vi "Get XNET Signal Names.vi"(6 "Add Info?":bool, 7 "Parent Ref in":T1 format="%.0x", 8 "error in":errorcluster, 9 "Tree In":refnum<vi>, 10 "XNET Cluster":refnum<k21>) -> (0 "error out":errorcluster, 1 "Tree Out":refnum<vi>, 3 "XNET Signal Names":refnum<k21>[](array[refnum]))   [LabVIEW 2025, in "Protection and Counter Addon System Explorer.lvlib"]
uses:
  Protection and Counter Addon System Explorer.lvlib
  <vilib>/NI VeriStand/Custom Device API/Custom Device Item Ref.ctl
  Types/Frame Tree and Database Pairing.ctl
  <vilib>/NI VeriStand/Custom Device API/Custom Device Channel.ctl
  <vilib>/NI VeriStand/Custom Device API/Custom Device Channel Type.ctl
  <vilib>/xnet/xnet.llb/XNET Get DBC Mode.ctl
  Addon Shared/SubVIs/GUID Lookup.vi
  <vilib>/NI VeriStand/Custom Device Tools/Custom Device Utility Library/NI VeriStand - Search for Item by Name.vi
  <vilib>/NI VeriStand/Custom Device API/Set Item Property (U32).vi
  <vilib>/xnet/xnet.llb/XNET Database Get DBC Attribute (Signal).vi
  <resource>/objmgr/xnet.rc
  <vilib>/NI VeriStand/Custom Device API/Custom Device API.lvlib
  Addon Shared/Protection and Counter Addon Shared.lvlib
  <vilib>/NI VeriStand/Custom Device Tools/Custom Device Utility Library/Custom Device Utility Library.lvlib
  <vilib>/NI/NI VeriStand Advanced SysDef API/SysDef API/Advanced System Definition.lvlib
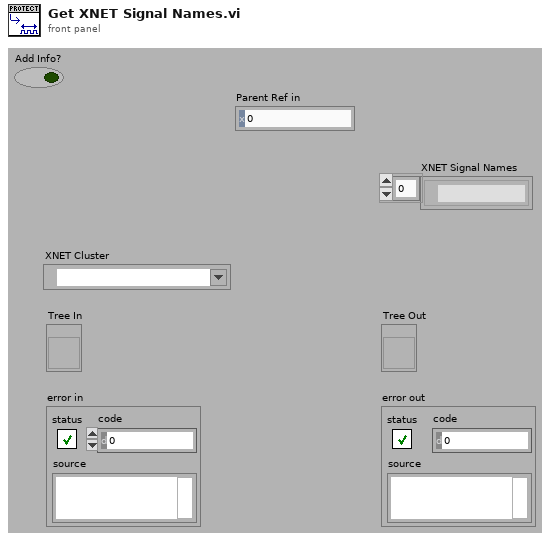
[diagram p1: front panel]
types:
  T1 = typedef "Custom Device API.lvlib/Custom Device Item Ref.ctl" = u64
  T2 = typedef "Protection and Counter Addon System Explorer.lvlib/Frame Tree and Database Pairing.ctl" = cluster{"Tree Tag":string, "Database Tag":string}
  T3 = typedef "Custom Device API.lvlib/Custom Device Channel.ctl" = cluster{"Type":T4, "Units":string, "Default Value":dbl, "Faultable":bool, "Scalable":bool}
  T4 = typedef "Custom Device API.lvlib/Custom Device Channel Type.ctl" = enum16{"Input", "Output"}
  T5 = typedef "Custom Device API.lvlib/Custom Device Item Info.ctl" = cluster{"Name":string, "Is Channel":bool, "GUID":string, "Is Waveform":bool}
  T6 = typedef "XNET Get DBC Mode.ctl" = u32
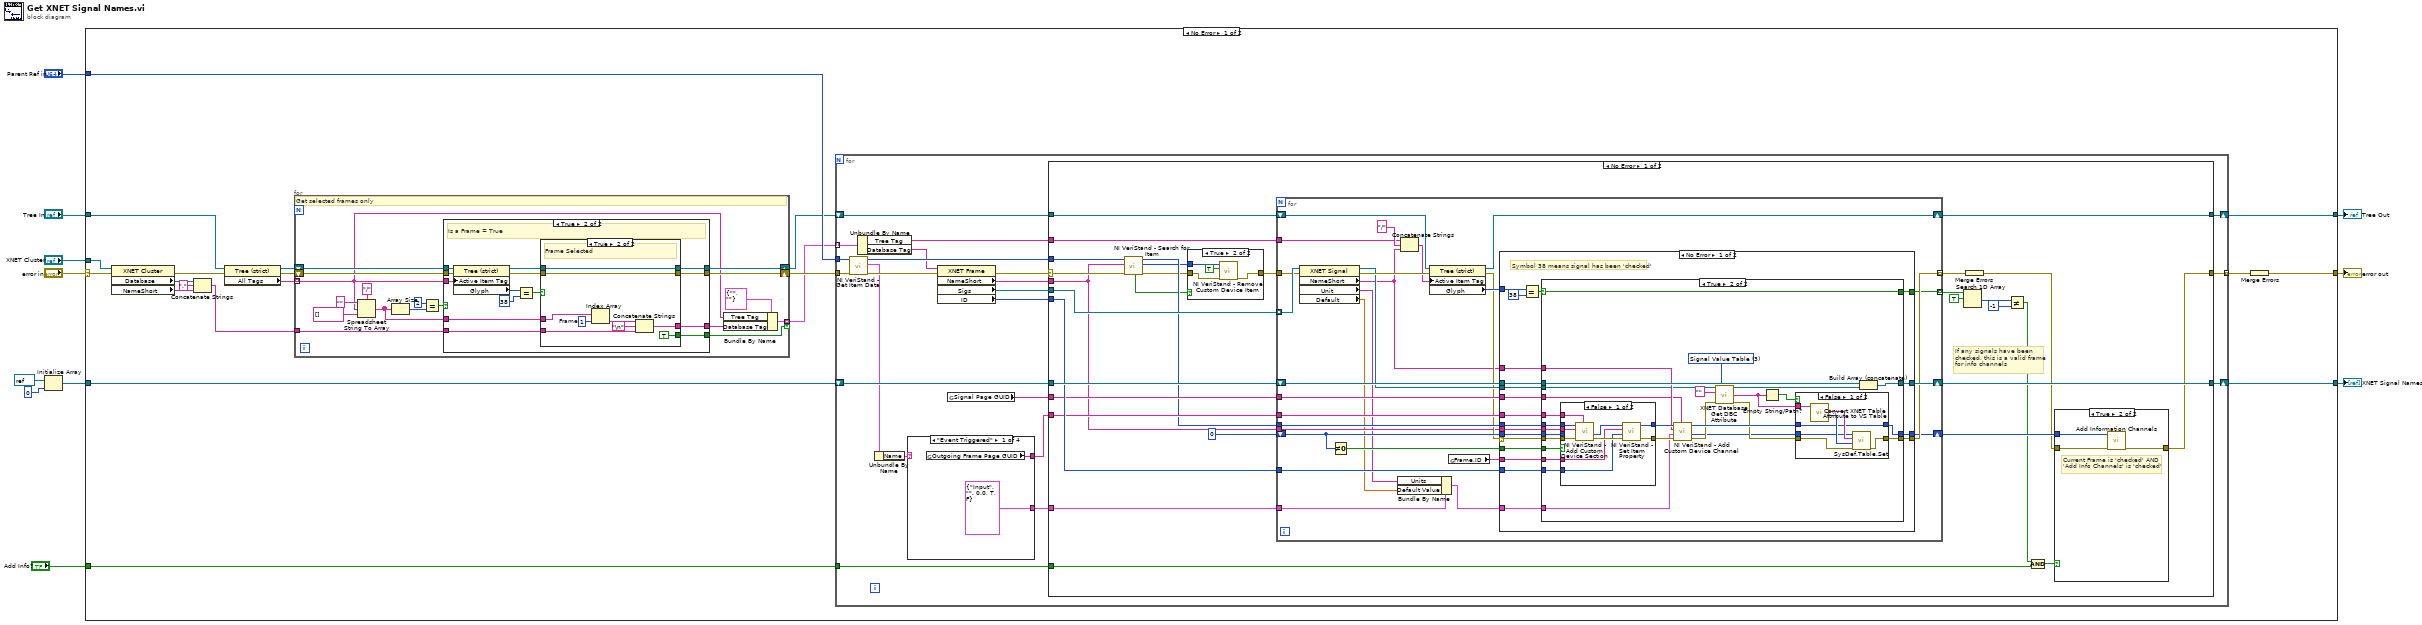
[diagram p0: block diagram]
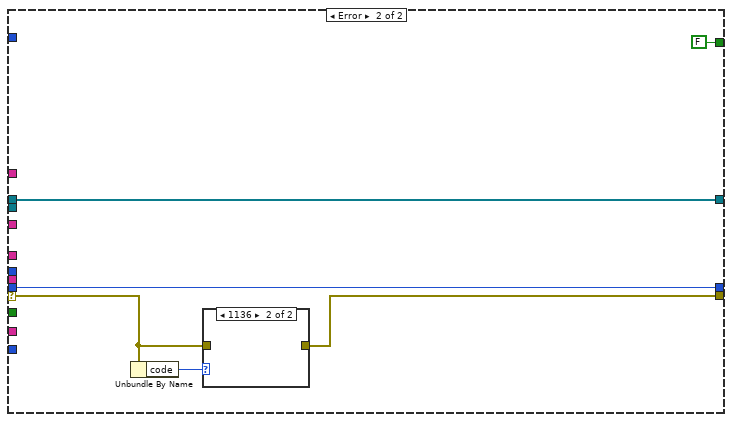
[diagram p7: hidden frame]
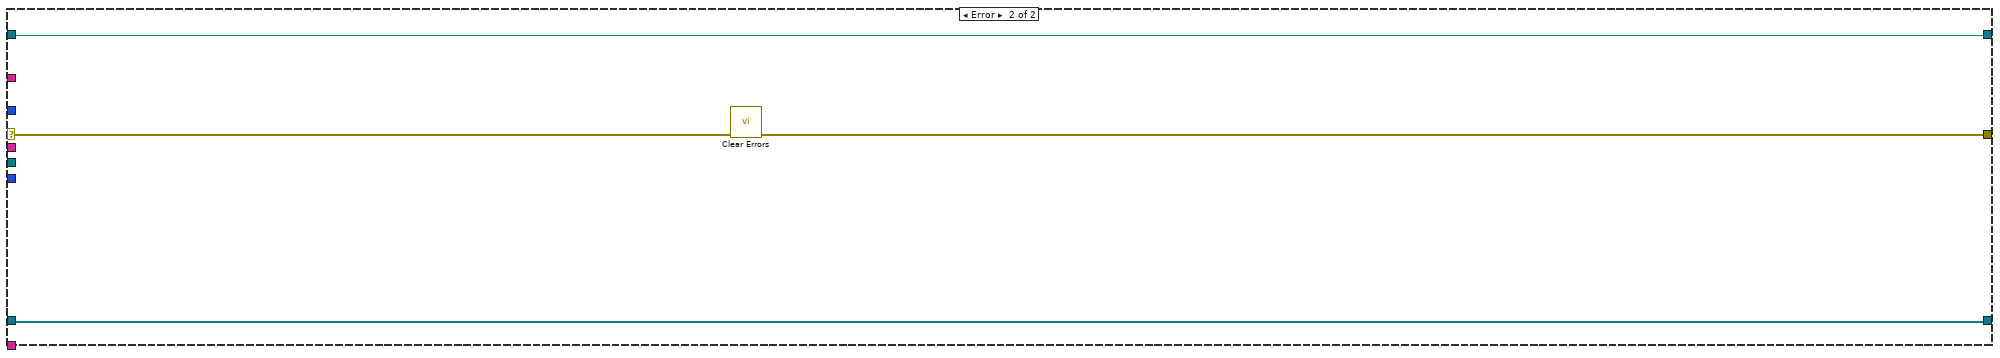
[diagram p11: hidden frame]
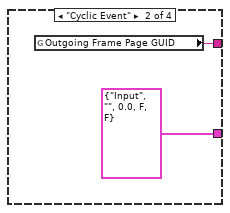
[diagram p12: hidden frame]
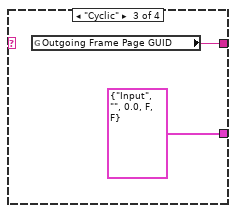
[diagram p13: hidden frame]
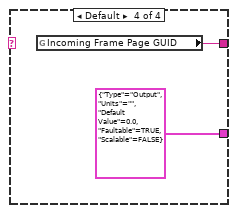
[diagram p14: hidden frame]
diagram:
  n1 = Initialize Array(refnum<k21> refnum ("XNET Signal"), 0 ("dimension size")) -> (w7:refnum<k21>[])
  n2 = case shown="No Error" "error in" {
    selector: "error in" -> [w23 w260]
    tunnel: "XNET Cluster" -> [w20 _]
    tunnel: [w12 w260] -> w2
    tunnel: [w31 _] -> w9
    tunnel: w7 -> [w30 _]
    tunnel: "Tree In" -> [w24 w259]
    tunnel: [w29 w259] -> w5
    tunnel: "Parent Ref in" -> [w28 _]
    tunnel: "Add Info?" -> [w27 _]
    frame No Error {
      n3 = property class="XNET Cluster"(reference=w20, error in=w23) -> (error out=w21:errorcluster, "Database"=w19:refnum<k21>, "NameShort"=w17:string)  [unwired: 1 out]
      n4 = Concatenate Strings(w19, "." ("string"), w17) -> (w15:string)
      n5 = property class="Tree (strict)"(reference=w24, error in=w21) -> (reference out=w25:refnum<vi>, error out=w22:errorcluster, "All Tags"=w26:string[])
      n6 = for {
        tunnel: w26 -> [w34] mode=indexing
        tunnel: [w33] -> w13 mode=indexing if=w40
        shift-right: [w43] -> w16
        shift-left: w25 -> [w44]
        shift-right: [w39] -> w14
        shift-left: w22 -> [w42]
        tunnel: w15 -> [w38]
        # "Get selected frames only"
        n7 = Spreadsheet String To Array(delimiter (Tab)="/", format string="", spreadsheet string=w34, array type (2D Dbl)=string[] [] ("All Tags")) -> (array=w37:string[])
        n8 = Array Size(array=w37) -> (size(s)=w46:i32)
        n9 = Equal?(x=2, y=w46) -> (x = y?=w41:bool)
        n10 = case shown="True" w41 {
          tunnel: w44 -> [w51 w65]
          tunnel: [w51 w55] -> w43
          tunnel: [_ w52] -> w40
          tunnel: w34 -> [_ w62]
          tunnel: w42 -> [w50 w61]
          tunnel: [w50 w54] -> w39
          tunnel: w38 -> [_ w58]
          tunnel: w37 -> [_ w57]
          tunnel: [_ w53] -> w36
          frame False {
            # "Not a Frame"
          }
          frame True {
            # "Is a Frame = True"
            n11 = property class="Tree (strict)"(reference=w65, error in=w61, "Active Item Tag"=w62) -> (reference out=w56:refnum<vi>, error out=w60:errorcluster, "Glyph"=w64:i32)
            n12 = Equal?(x=w64, y=38) -> (x = y?=w59:bool)
            n13 = case shown="True" w59 {
              tunnel: w60 -> [w67 w70]
              tunnel: w58 -> [_ w72]
              tunnel: w57 -> [_ w76]
              tunnel: w56 -> [w66 w71]
              tunnel: [w66 w71] -> w55
              tunnel: [w67 w70] -> w54
              tunnel: [_ w69] -> w53
              tunnel: [_ TRUE] -> w52
              frame False {
                # "Frame not selected"
              }
              frame True {
                w75 = 1  # Frame
                # "Frame Selected"
                n14 = Index Array(array=w76, index=w75) -> (element=w74:string)
                n15 = Concatenate Strings(w74, "\n", w72) -> (w69:string)
              }
            }
          }
        }
        n16 = Bundle By Name(cluster=T2 {"Tree Tag"="", "Database Tag"=""}, "Tree Tag"=w34, "Database Tag"=w36) -> (w33:T2)
      }
      n17 = for {
        tunnel: w13 -> [w80] mode=indexing
        shift-right: [w95] -> w31
        shift-left: w30 -> [w96]
        shift-right: [w94] -> w29
        shift-left: w16 -> [w97]
        tunnel: w28 -> [w90]
        tunnel: w27 -> [w81]
        tunnel: w14 -> [w92]
        tunnel: [w98] -> w32 mode=indexing
        n18 = call <vilib>:"NI VeriStand - Get Item Data.vi"("error in (no error)"=w92, "Item Ref in"=w90) -> ("error out"=w91:errorcluster, "Item Info"=w88:T5, "Item Ref out"=w89:T1)  [unwired: 7 out]
        n19 = Unbundle By Name(w80) -> ("Tree Tag"=w78:string, "Database Tag"=w79:string)
        n20 = Unbundle By Name(w88) -> ("Name"=w87:string)
        n21 = case shown="\"Event Triggered\"" w87 {
          tunnel: [T3 {"Type"=enum."Input", "Units"="", "Default Value"=0.0, "Faultable"=TRUE, "Scalable"=FALSE} ("Channel") T3 {"Type"=enum."Input", "Units"="", "Default Value"=0.0, "Faultable"=FALSE, "Scalable"=FALSE} ("Channel") T3 {"Type"=enum."Input", "Units"="", "Default Value"=0.0, "Faultable"=FALSE, "Scalable"=FALSE} ("Channel") T3 {"Type"=enum."Output", "Units"="", "Default Value"=0.0, "Faultable"=TRUE, "Scalable"=FALSE} ("Channel")] -> w86
          tunnel: [w251 w253 w255 w257] -> w83
          frame "Event Triggered" {
            n22 = global read "GUID Lookup.vi" "Outgoing Frame Page GUID"() -> (w251:string)
          }
          frame "Cyclic Event" {
            n23 = global read "GUID Lookup.vi" "Outgoing Frame Page GUID"() -> (w253:string)
          }
          frame "Cyclic" {
            n24 = global read "GUID Lookup.vi" "Outgoing Frame Page GUID"() -> (w255:string)
          }
          frame Default {
            n25 = global read "GUID Lookup.vi" "Incoming Frame Page GUID"() -> (w257:string)
          }
        }
        n26 = property class="XNET Frame"(reference=w79, error in=w91) -> (error out=w93:errorcluster, "NameShort"=w85:string, "Sigs"=w77:refnum<k21>[], "ID"=w84:u32)  [unwired: 1 out]
        n27 = global read "GUID Lookup.vi" "Signal Page GUID"() -> (w82:string)
        n28 = case shown="No Error" w93 {
          selector: w93 -> [w102 w247]
          tunnel: w77 -> [w128 _]
          tunnel: w85 -> [w99 _]
          tunnel: [w120 w248] -> w98
          tunnel: w97 -> [w103 w249]
          tunnel: w96 -> [w127 w250]
          tunnel: [w126 w250] -> w95
          tunnel: [w119 w249] -> w94
          tunnel: w89 -> [w121 _]
          tunnel: w84 -> [w125 _]
          tunnel: w82 -> [w124 _]
          tunnel: w83 -> [w123 _]
          tunnel: w86 -> [w122 _]
          tunnel: w81 -> [w118 _]
          tunnel: w78 -> [w101 _]
          frame No Error {
            # "If any signals have been\nchecked, this is a valid frame\nfor info channels"
            n29 = call-poly <vilib>:"NI VeriStand - Search for Item.vi"("error in"=w102, "Item Name"=w99, "Section Ref in"=w121) -> ("error out"=w113:errorcluster, "Item Ref"=w114:T1, "Section Ref out"=w116:T1, "Found"=w115:bool)  [unwired: 5 in]
            n30 = case shown="True" w115 {
              tunnel: w114 -> [_ w242]
              tunnel: w113 -> [w238 w241]
              tunnel: [w238 w240] -> w112
              frame False {
              }
              frame True {
                n31 = call <vilib>:"NI VeriStand - Remove Custom Device Item.vi"("error in (no error)"=w241, "Force Delete (F)"=TRUE, "Item Ref in"=w242) -> ("error out"=w240:errorcluster)  [unwired: 7 in, 1 out]
              }
            }
            n32 = for {
              tunnel: w128 -> [w157] mode=indexing
              tunnel: w101 -> [w138]
              shift-right: [w151] -> w126
              shift-left: w127 -> [w150]
              shift-right: [w148] -> w119
              shift-left: w103 -> [w153]
              tunnel: w116 -> [w146]
              shift-right: [w145] -> w111
              shift-left: T1 0 ("Parent Ref out") -> [w144]
              tunnel: w125 -> [w142]
              tunnel: w124 -> [w141]
              tunnel: w123 -> [w140]
              tunnel: w122 -> [w139]
              tunnel: [w134] -> w106 mode=indexing
              tunnel: w112 -> [w156]
              tunnel: [w147] -> w110 mode=indexing
              tunnel: w99 -> [w132]
              n33 = property class="XNET Signal"(reference=w157, error in=w156) -> (reference out=w149:refnum<k21>, error out=w154:errorcluster, "NameShort"=w133:string, "Unit"=w130:string, "Default"=w129:dbl)
              n34 = Not Equal To 0?(x=w144) -> (x != 0?=w143:bool)
              n35 = Bundle By Name(cluster=w139, "Units"=w130, "Default Value"=w129) -> (w131:T3)
              n36 = Concatenate Strings(w138, "/" ("string"), w133) -> (w135:string)
              n37 = property class="Tree (strict)"(reference=w153, error in=w154, "Active Item Tag"=w135) -> (reference out=w148:refnum<vi>, error out=w137:errorcluster, "Glyph"=w152:i32)
              n38 = global read "GUID Lookup.vi" "Frame.ID"() -> (w136:string)
              n39 = case shown="No Error" w137 {
                selector: w137 -> [w159 w233]
                tunnel: w152 -> [w177 _]
                tunnel: [w174 w235] -> w151
                tunnel: w150 -> [w173 w235]
                tunnel: w149 -> [w172 _]
                tunnel: [w171 w232] -> w147
                tunnel: w146 -> [w170 _]
                tunnel: [w169 w236] -> w145
                tunnel: w144 -> [w168 w236]
                tunnel: w143 -> [w167 _]
                tunnel: w133 -> [w166 _]
                tunnel: w142 -> [w165 _]
                tunnel: w136 -> [w164 _]
                tunnel: w141 -> [w163 _]
                tunnel: w140 -> [w162 _]
                tunnel: w131 -> [w161 _]
                tunnel: w132 -> [w160 _]
                tunnel: [w158 FALSE] -> w134
                frame No Error {
                  # "Symbol 38 means signal has been 'checked'"
                  n40 = Equal?(x=w177, y=38) -> (x = y?=w175:bool)
                  n41 = case shown="True" w175 {
                    selector: w175 -> [w178 w194]
                    tunnel: [w181 w208] -> w174
                    tunnel: w173 -> [w181 w209]
                    tunnel: w172 -> [_ w184]
                    tunnel: w167 -> [_ w207]
                    tunnel: w160 -> [_ w206]
                    tunnel: w159 -> [w180 w205]
                    tunnel: [w180 w192] -> w171
                    tunnel: w170 -> [_ w204]
                    tunnel: [w179 w191] -> w169
                    tunnel: w168 -> [w179 w203]
                    tunnel: w166 -> [_ w200]
                    tunnel: w162 -> [_ w199]
                    tunnel: w163 -> [_ w198]
                    tunnel: w165 -> [_ w197]
                    tunnel: w164 -> [_ w196]
                    tunnel: w161 -> [_ w195]
                    tunnel: [w178 w194] -> w158
                    frame False {
                    }
                    frame True {
                      w188 = T6 3 items=["Attribute Value", "Enumeration", "Attribute Name List", "Signal Value Table"] ("mode")
                      n42 = case shown="False" w207 {
                        tunnel: w206 -> [w228 _]
                        tunnel: w205 -> [w227 w230]
                        tunnel: [w220 w230] -> w202
                        tunnel: w204 -> [w226 _]
                        tunnel: [w219 w229] -> w201
                        tunnel: w203 -> [_ w229]
                        tunnel: w199 -> [w225 _]
                        tunnel: w197 -> [w221 _]
                        tunnel: w196 -> [w222 _]
                        frame False {
                          n43 = call <vilib>:"NI VeriStand - Add Custom Device Section.vi"("GUID (Default Section)"=w225, "error in (no error)"=w227, "Section Name"=w228, "Parent Ref in"=w226) -> ("error out"=w223:errorcluster, "Section Ptr"=w224:T1)  [unwired: 4 in, 2 out]
                          n44 = call-poly <vilib>:"NI VeriStand - Set Item Property.vi"("error in (no error)"=w223, "Value"=w221, "Property Name"=w222, "Item Ref in"=w224) -> ("error out"=w220:errorcluster, "Item Ref out"=w219:T1)  [unwired: 5 in, 1 out]
                        }
                        frame True {
                        }
                      }
                      n45 = call <vilib>:"NI VeriStand - Add Custom Device Channel.vi"("GUID (Default Channel)"=w198, "error in (no error)"=w202, "Channel"=w195, "Channel Name"=w200, "Parent Ref in"=w201) -> ("error out"=w190:errorcluster, "Channel Ref"=w182:T1, "Parent Ref out"=w193:T1)  [unwired: 3 in, 1 out]
                      n46 = call-poly <vilib>:"XNET Database Get DBC Attribute.vi"("signal in"=w184, "mode"=w188, "attribute name"="", "error in (no error)"=w190) -> ("signal out"=w185:refnum<k21>, "attribute text"=w183:string, "error out"=w189:errorcluster)  [unwired: 8 in, 1 out]
                      n47 = Empty String/Path?(string/path=w183) -> (empty?=w186:bool)
                      n48 = case shown="False" w186 {
                        tunnel: w193 -> [w210 w218]
                        tunnel: [w216 w217] -> w192
                        tunnel: [w210 w218] -> w191
                        tunnel: w189 -> [w215 w217]
                        tunnel: w183 -> [w214 _]
                        tunnel: w182 -> [w211 _]
                        frame False {
                          n49 = call "Convert XNET Table Attribute to VS Table.vi"("attribute text"=w214) -> ("Value"=w212:i64[], "Names"=w213:string[])  [unwired: 9 in]
                          n50 = call <vilib>:"SysDef.Table.Set.vi"("error in (no error)"=w215, "Values"=w212, "Names"=w213, "nodeID"=w211) -> ("error out"=w216:errorcluster)  [unwired: 6 in, 1 out]
                        }
                        frame True {
                        }
                      }
                      n51 = Build Array (concatenate)(w209, w185) -> (w208:refnum<k21>[])
                    }
                  }
                }
                frame Error {
                  n52 = Unbundle By Name(w233) -> ("code"=w234:i32)
                  n53 = case shown="1136" w234 {
                    tunnel: [w237 _] -> w232
                    tunnel: w233 -> [w237 _]
                    frame Default {
                    }
                    frame 1136 {
                    }
                  }
                }
              }
            }
            n54 = Search 1D Array(1D array=w106, element=TRUE) -> (index of element=w104:i32)  [unwired: 1 in]
            n55 = Merge Errors(w110) -> (w100:errorcluster)
            n56 = Not Equal?(x=w104, y=-1) -> (x != y?=w108:bool)
            n57 = Compound Arithmetic op=AND(w108, w118) -> (w109:bool)
            n58 = case shown="True" w109 {
              tunnel: w111 -> [_ w246]
              tunnel: w100 -> [w243 w245]
              tunnel: [w243 w244] -> w120
              frame False {
              }
              frame True {
                # "Current Frame is 'checked' AND\n'Add Info Channels' is 'checked'"
                n59 = call "Add Information Channels.vi"("error in (no error)"=w245, "Node Ptr"=w246) -> ("error out"=w244:errorcluster)  [unwired: 8 in, 1 out]
              }
            }
          }
          frame Error {
            n60 = call <vilib>:"Clear Errors.vi"("error in (no error)"=w247) -> ("error out"=w248:errorcluster)  [unwired: 5 in, 1 out]
          }
        }
      }
      n61 = Merge Errors(w32) -> (w12:errorcluster)
    }
    frame Error {
    }
  }
  "error out" <- w2
  "XNET Signal Names" <- w9
  "Tree Out" <- w5
